vi "Handle Value Change.vi"(5 "VolatusAPI":refnum<class "VolatusAPI.lvclass">, 7 "CtlRef":refnum<vi>, 8 "error in (no error)":errorcluster, 9 "NewVal":variant, 10 "OldVal":variant, 11 "BooleanControl in":refnum<class "BooleanControl.lvclass">) -> (0 "error out":errorcluster, 3 "BooleanControl out":refnum<class "BooleanControl.lvclass">)   [LabVIEW 2020, in "VolatusGUIElements.lvlib" / "BooleanControl.lvclass"]
uses:
  BooleanControl.lvclass
  C:/dev/lv20CE/relink/lv-volatus/VolatusGUI/GUI Element/GUI Element.lvclass
  Volatus/VolatusAPI/VolatusAPI.lvclass
  BooleanControl.lvclass/BooleanControl.ctl
  messages/CmdDigital/Class/Msg.lvclass/Msg.ctl
  Volatus/VolatusAPI/VolatusAPI.lvclass/VolatusAPI.ctl
  messages/CmdDigital/Class/Msg.lvclass
  C:/dev/lv20CE/relink/lv-protoc/LV-Proto/Message/Message.lvclass
  lv-vecto/Vecto/TCPMessageService/Send Message.vi
  <vilib>/Utility/error.llb/Error Cluster From Error Code.vi
  lv-protoc/LV-Proto/Message/Message.lvclass
  VolatusGUI/GUI Element/GUI Element.lvclass
  Volatus/Digital Command/Digital Command.lvclass
  C:/dev/lv20CE/relink/lv-volatus/VolatusGUIElements/BooleanControl/BooleanControl.lvclass
  C:/dev/lv20CE/relink/lv-volatus/VolatusGUI/OnValueChangeHandler/OnValueChangeHandler.lvclass
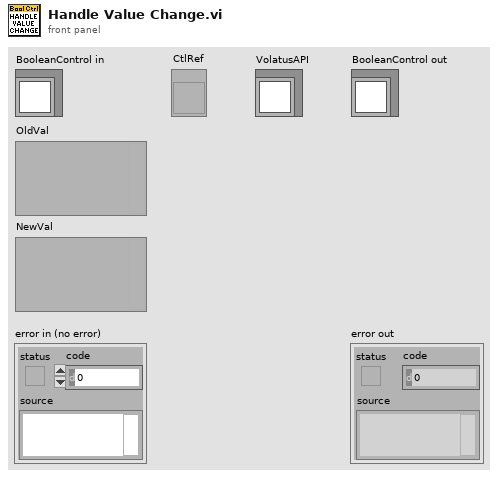
[diagram p1: front panel]
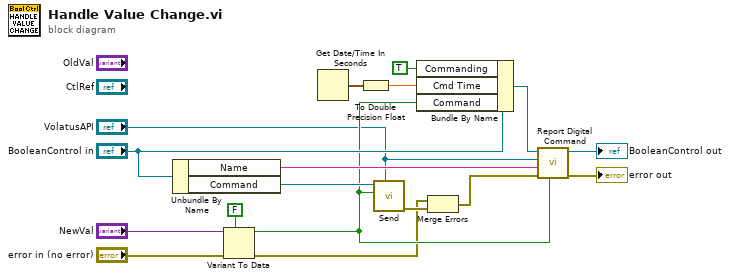
[diagram p0: block diagram]
diagram:
  n1 = Unbundle By Name("BooleanControl in") -> ("Name"=w12:string, "Command"=w6:refnum<class "Digital Command.lvclass">)
  n2 = Variant To Data(error in="error in (no error)", type=FALSE, Variant="NewVal") -> (data=w5:bool, error out=w1:errorcluster)
  n3 = Get Date/Time In Seconds() -> (seconds since 1Jan1904=w9:timestamp)
  n4 = To Double Precision Float(number=w9) -> (double precision float=w8:dbl)
  n5 = call "Send.vi"("VolatusAPI"="VolatusAPI", "Value"=w5, "Digital Command in"=w6) -> ("error out"=w3:errorcluster)  [unwired: 7 in, 1 out]
  n6 = Bundle By Name(cluster="BooleanControl in", "Commanding"=TRUE, "Cmd Time"=w8, "Command"=w5) -> (w10:refnum<class "BooleanControl.lvclass">)
  n7 = Merge Errors(w1, w3) -> (w2:errorcluster)
  n8 = call "Report Digital Command.vi"("Value"=w5, "error in (no error)"=w2, "Name"=w12, "VolatusAPI in"="VolatusAPI", "GUI Element in"=w10) -> ("error out"=→"error out":errorcluster, "GUI Element out"=→"BooleanControl out":refnum<class "BooleanControl.lvclass">)  [unwired: 5 in]
